vi "VIH Constant - Temporal Build Log File.vi"() -> (3 "Temporal Build Log File":path)   [LabVIEW 2014]
doc: "::: VI Helpeks :::\nCopyright (c) 2000-2026 Konstantin Shifershteyn. All rights reserved."
panel:
  # "VI Helpeks\nCopyright (c) 2012-2026 Konstantin Shifershteyn"
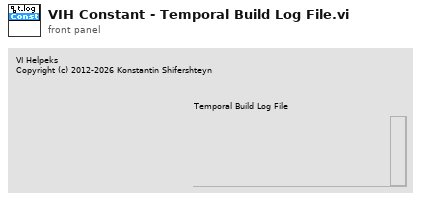
[diagram p1: front panel]
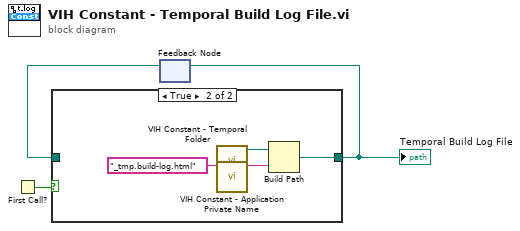
[diagram p0: block diagram]
diagram:
  n1 = First Call?() -> (First Call?: T/F=w3:bool)
  n2 = feedback #1() -> (w2:path)  [unwired: 1 in]
  n3 = case shown="True" w3 {
    tunnel: [w4 w5] -> w1
    tunnel: w2 -> [w4 _]
    frame False {
    }
    frame True {
      n4 = call "VIH Constant - Temporal Folder.vi"() -> ("Temporal folder"=w6:path)  [unwired: 11 in]
      n5 = call "VIH Constant - Application Private Name.vi"("Append to name"="_tmp.build-log.html") -> ("Name out"=w7:string)  [unwired: 10 in]
      n6 = Build Path(base path=w6, name or relative path=w7) -> (appended path=w5:path)
    }
  }
  "Temporal Build Log File" <- w1
  n7 = feedback-in #1(w1) -> ()
